vi "set Uplink Channel Number.vi"(8 "error in (no error)":errorcluster, 9 "UL Channel Arguments":T2, 10 "UL Channel Info":T1, 11 "LTE in":refnum<class "LTE.lvclass">) -> (0 "error out":errorcluster, 3 "LTE out":refnum<class "LTE.lvclass">)   [LabVIEW 2023, in "ANRITSU Call Box.lvlib" / "LTE.lvclass"]
uses:
  LTE.lvclass
  LTE.lvclass/LTE.ctl
  Type Definition/LTE Uplink Channel Number Target.ctl
  ANRITSU Call Box.lvlib
  Type Definition/LTE Uplink Channel Number Info.ctl
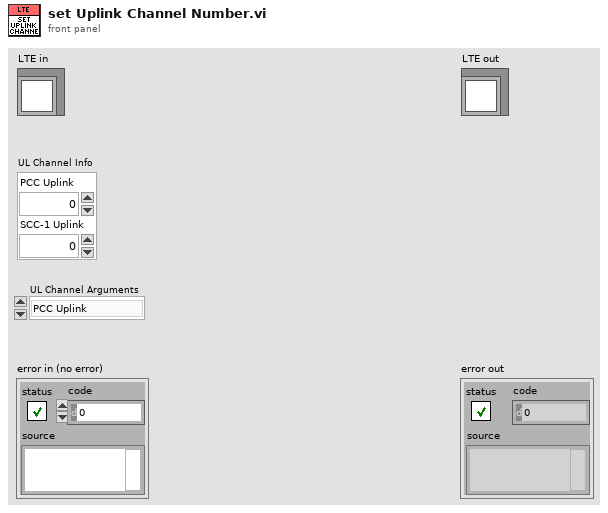
[diagram p1: front panel]
types:
  T1 = typedef "ANRITSU Call Box.lvlib/LTE Uplink Channel Number Info.ctl" = cluster{"PCC Uplink":i32, "SCC-1 Uplink":i32}
  T2 = typedef "ANRITSU Call Box.lvlib/LTE Uplink Channel Number Target.ctl" = enum16{"PCC Uplink", "SCC-1 Uplink", "All"}
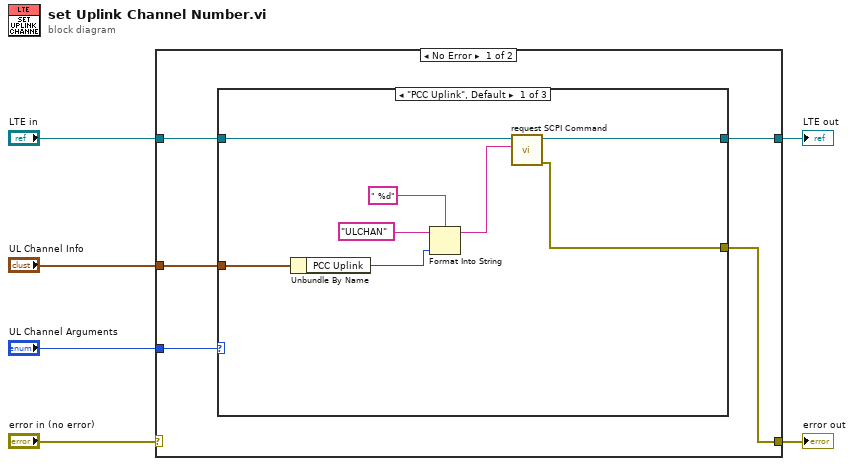
[diagram p0: block diagram]
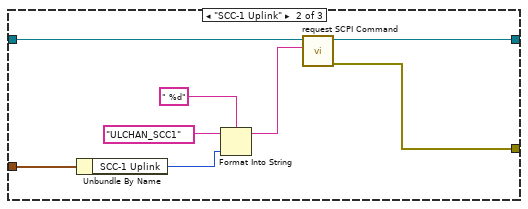
[diagram p2: hidden frame]
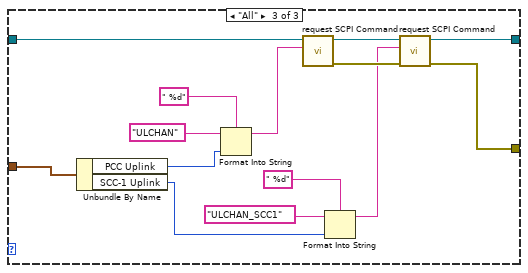
[diagram p3: hidden frame]
diagram:
  n1 = case shown="No Error" "error in (no error)" {
    selector: "error in (no error)" -> [_ w43]
    tunnel: [w7 w43] -> w5
    tunnel: [w8 w42] -> w3
    tunnel: "LTE in" -> [w9 w42]
    tunnel: "UL Channel Arguments" -> [w11 _]
    tunnel: "UL Channel Info" -> [w10 _]
    frame No Error {
      n2 = case shown="\"PCC Uplink\", Default" w11 {
        tunnel: w10 -> [w18 w26 w40]
        tunnel: w9 -> [w19 w27 w41]
        tunnel: [w13 w22 w34] -> w8
        tunnel: [w12 w20 w32] -> w7
        frame "PCC Uplink", Default {
          n3 = Unbundle By Name(w18) -> ("PCC Uplink"=w15:i32)
          n4 = Format Into String(format string=" %d", initial string="ULCHAN" ("string"), w15) -> (resulting string=w14:string)  [unwired: 1 in, 1 out]
          n5 = call "request SCPI Command.vi"("SCPI Command"=w14, "LTE in"=w19) -> ("error out"=w12:errorcluster, "LTE out"=w13:refnum<class "LTE.lvclass">)  [unwired: 8 in]
        }
        frame "SCC-1 Uplink" {
          n6 = Unbundle By Name(w26) -> ("SCC-1 Uplink"=w24:i32)
          n7 = Format Into String(format string=" %d", initial string="ULCHAN_SCC1" ("string"), w24) -> (resulting string=w23:string)  [unwired: 1 in, 1 out]
          n8 = call "request SCPI Command.vi"("SCPI Command"=w23, "LTE in"=w27) -> ("error out"=w20:errorcluster, "LTE out"=w22:refnum<class "LTE.lvclass">)  [unwired: 8 in]
        }
        frame "All" {
          n9 = Unbundle By Name(w40) -> ("PCC Uplink"=w37:i32, "SCC-1 Uplink"=w30:i32)
          n10 = Format Into String(format string=" %d", initial string="ULCHAN" ("string"), w37) -> (resulting string=w36:string)  [unwired: 1 in, 1 out]
          n11 = call "request SCPI Command.vi"("SCPI Command"=w36, "LTE in"=w41) -> ("error out"=w33:errorcluster, "LTE out"=w35:refnum<class "LTE.lvclass">)  [unwired: 8 in]
          n12 = Format Into String(format string=" %d", initial string="ULCHAN_SCC1" ("string"), w30) -> (resulting string=w28:string)  [unwired: 1 in, 1 out]
          n13 = call "request SCPI Command.vi"("error in (no error)"=w33, "SCPI Command"=w28, "LTE in"=w35) -> ("error out"=w32:errorcluster, "LTE out"=w34:refnum<class "LTE.lvclass">)  [unwired: 7 in]
        }
      }
    }
    frame Error {
    }
  }
  "error out" <- w5
  "LTE out" <- w3
